vi "Persistent_MakePersistent.vi"(7 "Action":T1=enum."GeneratePattern", 8 "error in (no error)":errorcluster, 10 "DataIn":variant, 11 "ClassRefToActOn":refnum<vi>) -> (0 "error out":errorcluster, 1 "Name":string, 2 "DataOut":variant, 3 "Cancelled":bool)   [LabVIEW 2020]
uses:
  Provider_BaseClassInterface/BaseProvider_SubVIs/BaseProvider_DesignPatternsActions.ctl
  Common/LvClass_class/GDSLvClass_ProviderTypes.ctl
  Provider_EndevoGOOP400/EndevoG4ProviderName.ctl
  <vilib>/picture/picture.llb/imagedata.ctl
  <vilib>/Utility/miscctls.llb/LVPositionTypeDef.ctl
panel:
  in  "StartAsPersitent":bool
  in  "_Cancel":bool
  in  "_OK":bool
  # "Persistent"
  # "This option will add an input to the New.vi that can make the objects persistent."
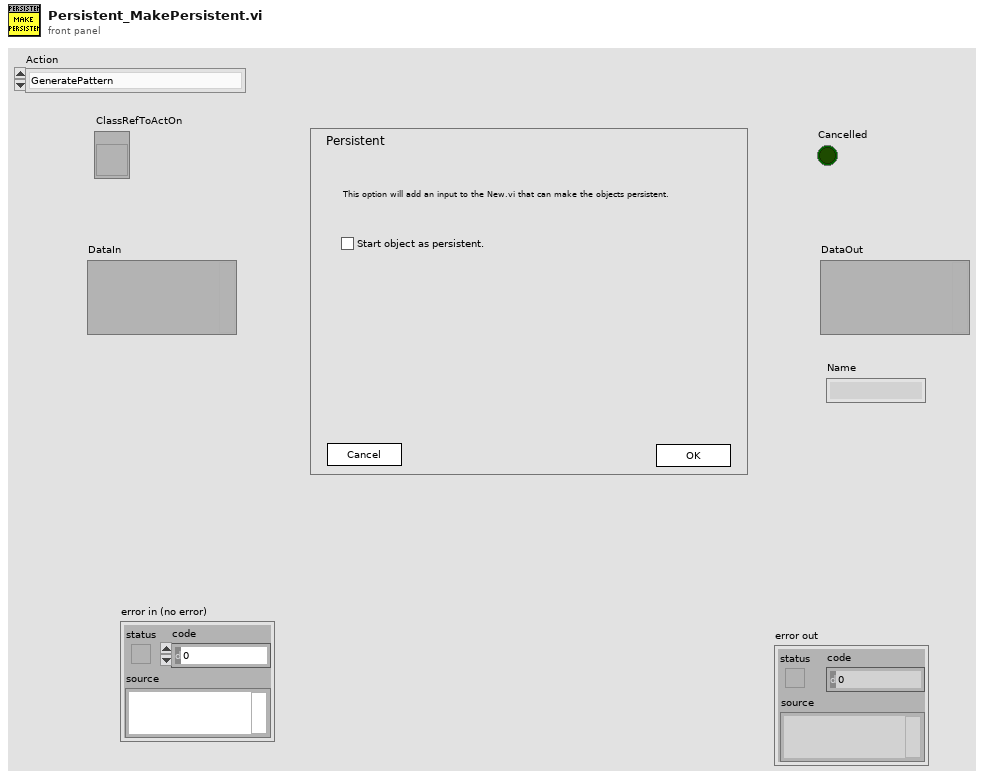
[diagram p1: front panel]
types:
  T1 = typedef "BaseProvider_DesignPatternsActions.ctl" = enum16{"AddPatternDialog", "GeneratePattern", "RemovePattern", "CreatePatternMethod", "UpdatePattern"}
  T2 = typedef "GDSLvClass_ProviderTypes.ctl" = enum16{"UnKnown(LabVOOP)", "Native", "EndevoGOOP3", "OpenG(RootObject)", "OpenG(OpenG_Object)", "EndevoGOOP4", "JKI1"}
  T3 = cluster{"Application":refnum<vi>, "SupportFolder":path, "TemplateName":string, "ClassProvider":T2, "UtilsFolder":path, "UtilsFolderRef":refnum<vi>, "ClassName":string, "Persistent_New.vi":path, "Persistent_CreateReference.vi":path, "NewRef":refnum<vi>, "CreateReferenceRef":refnum<vi>, "ProcessIdRef":refnum<vi>, "TemplateNewRef":refnum<vi>, "StartAsPersitent":bool, "PersistentCPIndex":i32, "FullClassName":string}
  T4 = cluster{"Cancelled":bool, "ClassPath":path, "DataOut":variant, "ClassName":string}
  T5 = typedef "EndevoG4ProviderName.ctl" = enum16{"EndevoGOOP400"}
  T6 = enum32{"invalid lock state", "Not Locked", "Locked (No Password)", "Password-protected"}
  T7 = typedef "LVPositionTypeDef.ctl" = cluster{"Left":i32, "Top":i32}
  T8 = typedef "imagedata.ctl" = cluster{"image type":i32, "image depth":i32, "image":u8[], "mask":u8[], "colors":u32[], "Rectangle":cluster{"left":i16, "top":i16, "right":i16, "bottom":i16}}
  T9 = typedef "GDSLvCLass_ClassSettingsType.ctl" = cluster{"ClassProviderName":string, "ClassTemplateUsed":string, "ClassTemplateVersion":string, "ClassDescription":string, "PlugIns":T10[], "ConnectorPanePattern":string}
  T10 = typedef "GDSLvClass_PlugIn.ctl" = cluster{"Type":T11, "ID":string, "Version":string, "Path":path, "Name":string, "Data":variant}
  T11 = typedef "GDSLvClass_PlugInTypes.ctl" = enum16{"DesignPattern", "MethodTypes"}
  T12 = typedef "GOOP400_Options.ctl" = cluster{"FlatFolderStructure":bool}
  T13 = typedef "GDSLvClass_IconSettingsType.ctl" = cluster{"Frame":u32, "Frame thickness":u8, "Header Background":u32, "Header Text":u32, "ColorPublic":u32, "ColorProtected":u32, "ColorPrivate":u32, "Body Text":u32, "ClassBodyIcon":string}
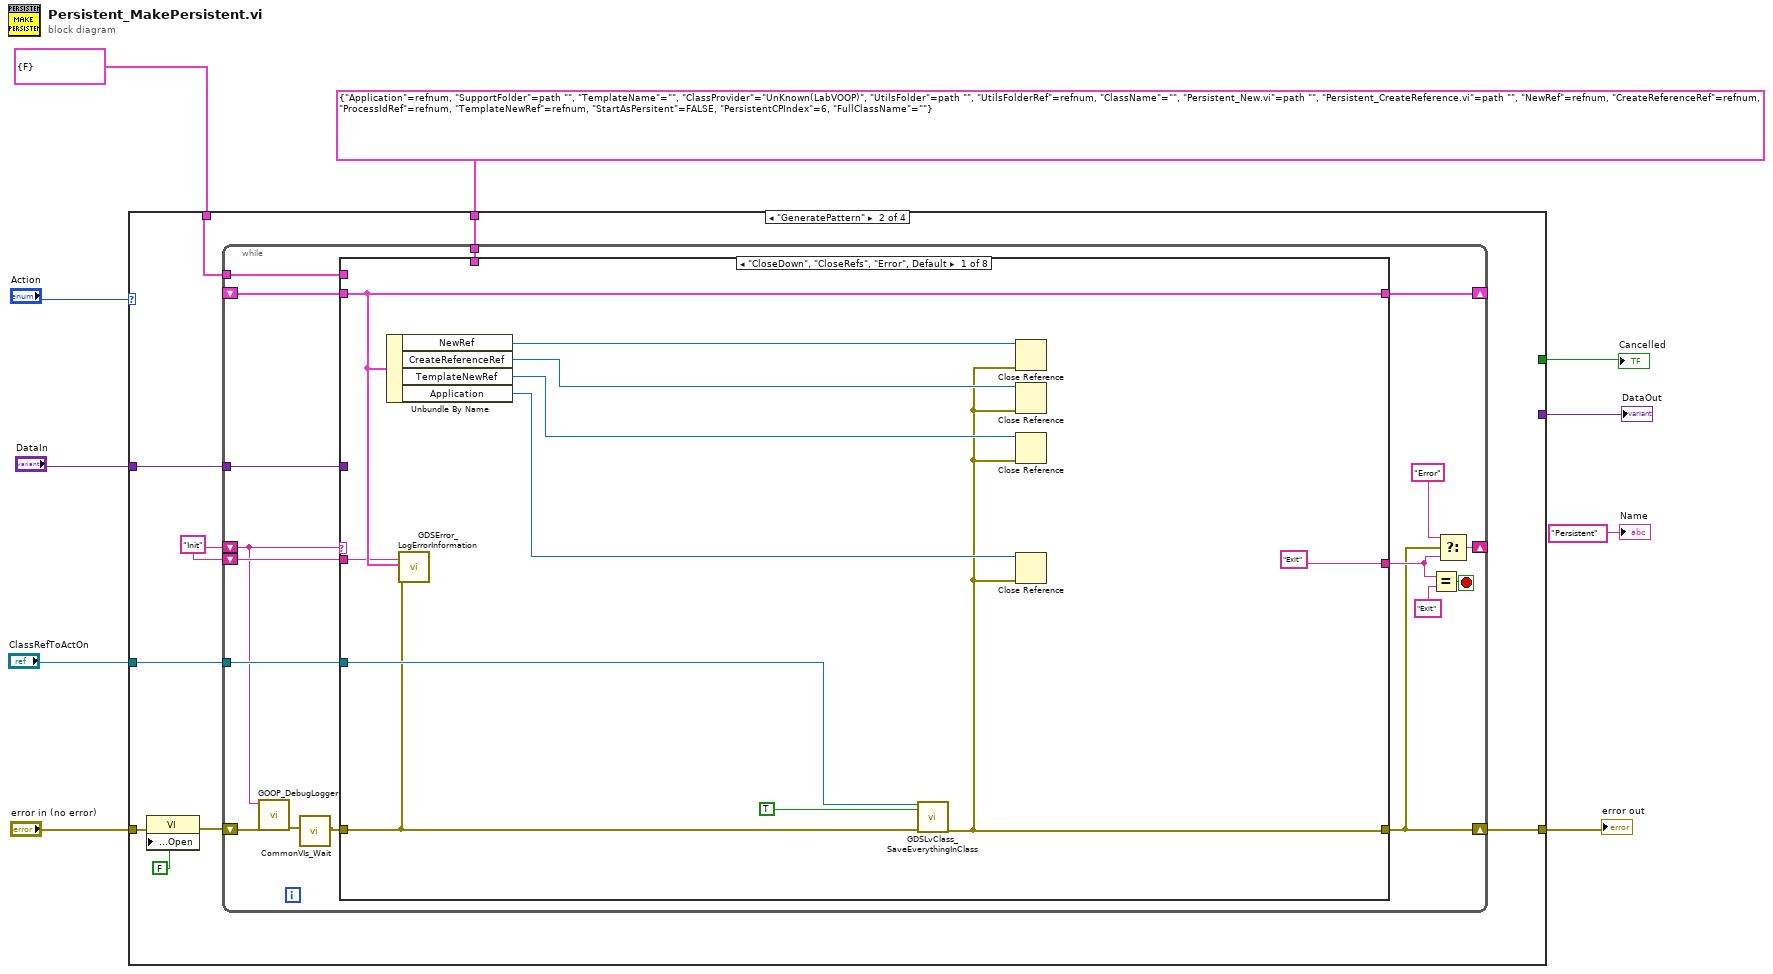
[diagram p0: block diagram]
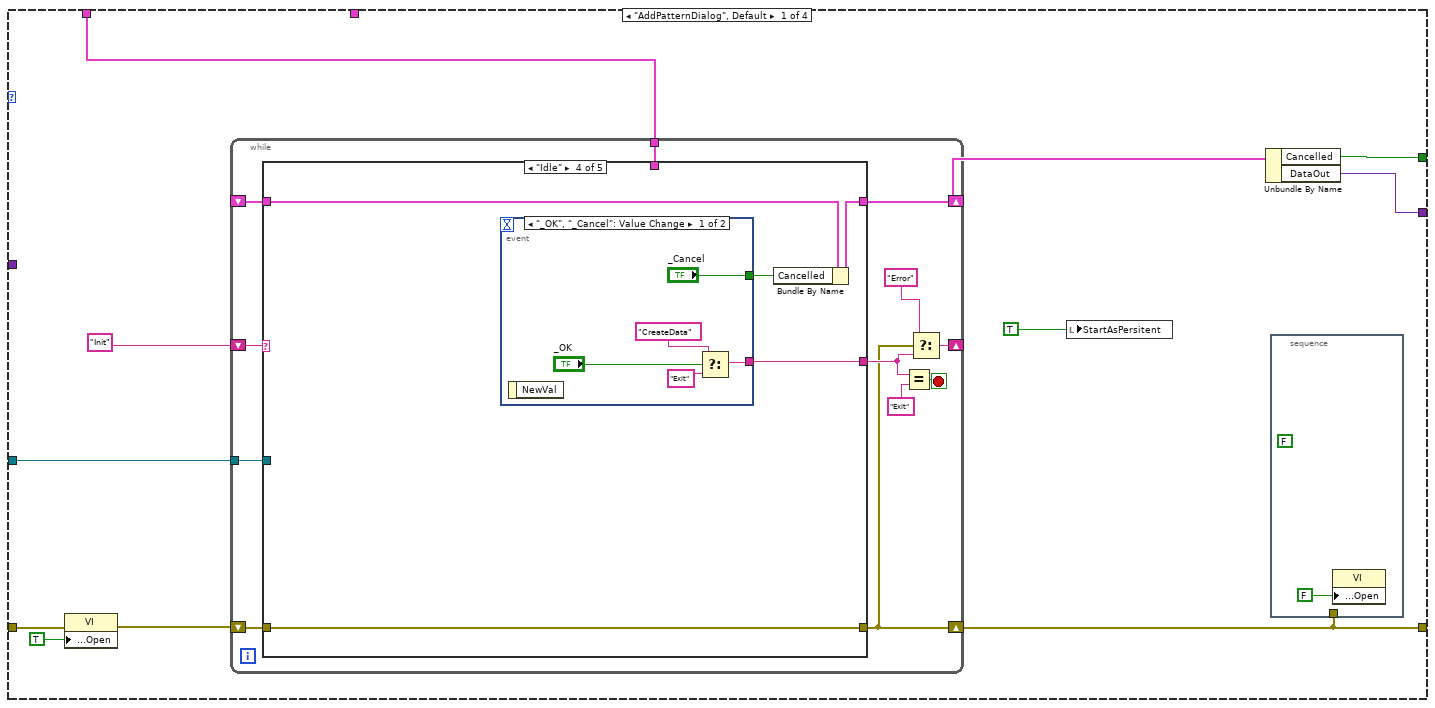
[diagram p2: hidden frame]
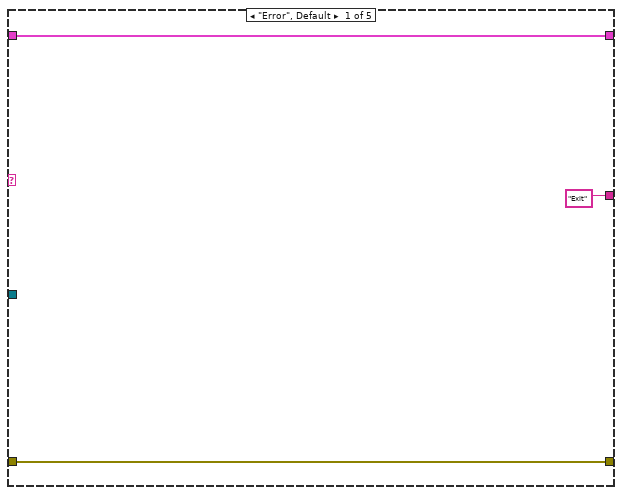
[diagram p3: hidden frame]
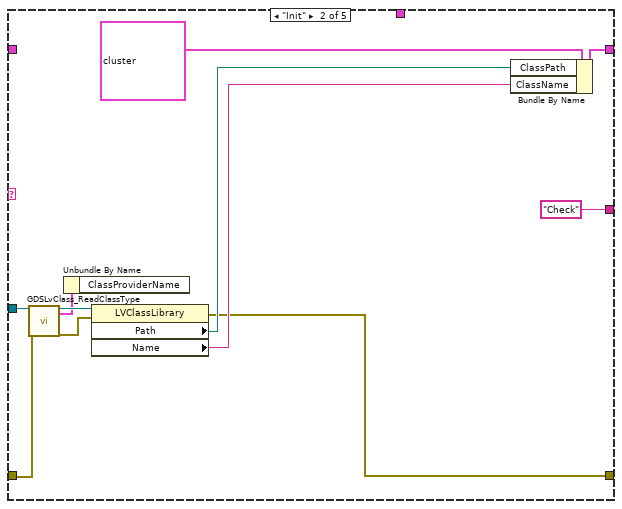
[diagram p4: hidden frame]
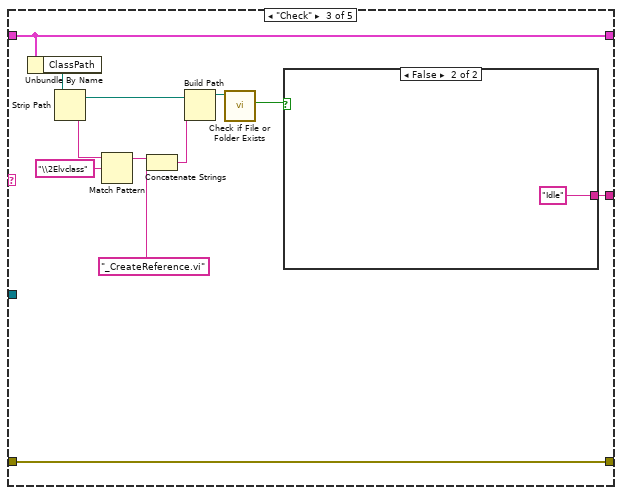
[diagram p5: hidden frame]
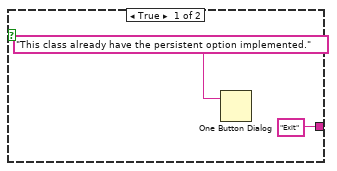
[diagram p6: hidden frame]
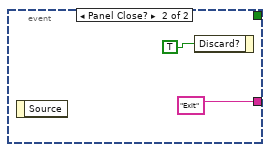
[diagram p7: hidden frame]
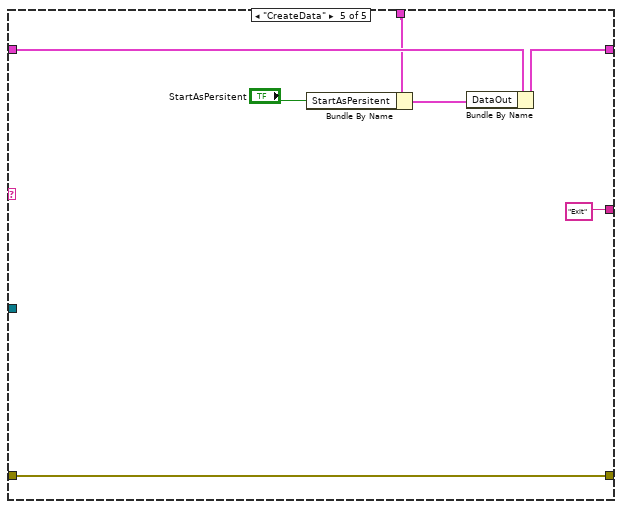
[diagram p8: hidden frame]
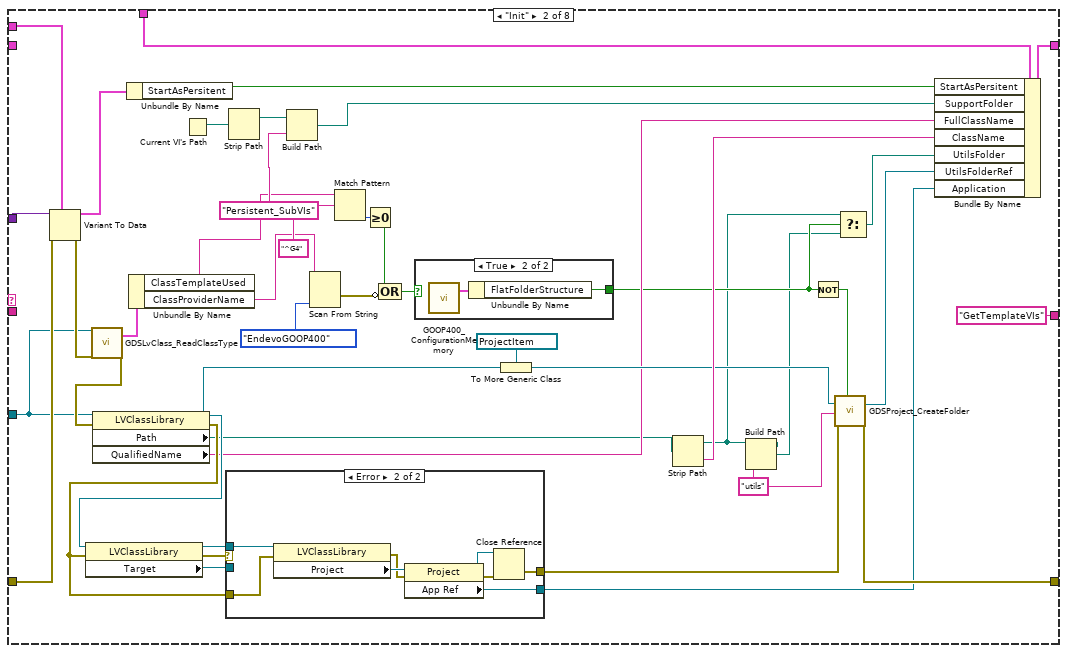
[diagram p9: hidden frame]
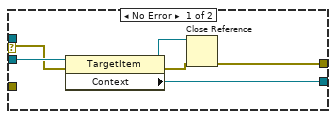
[diagram p11: hidden frame]
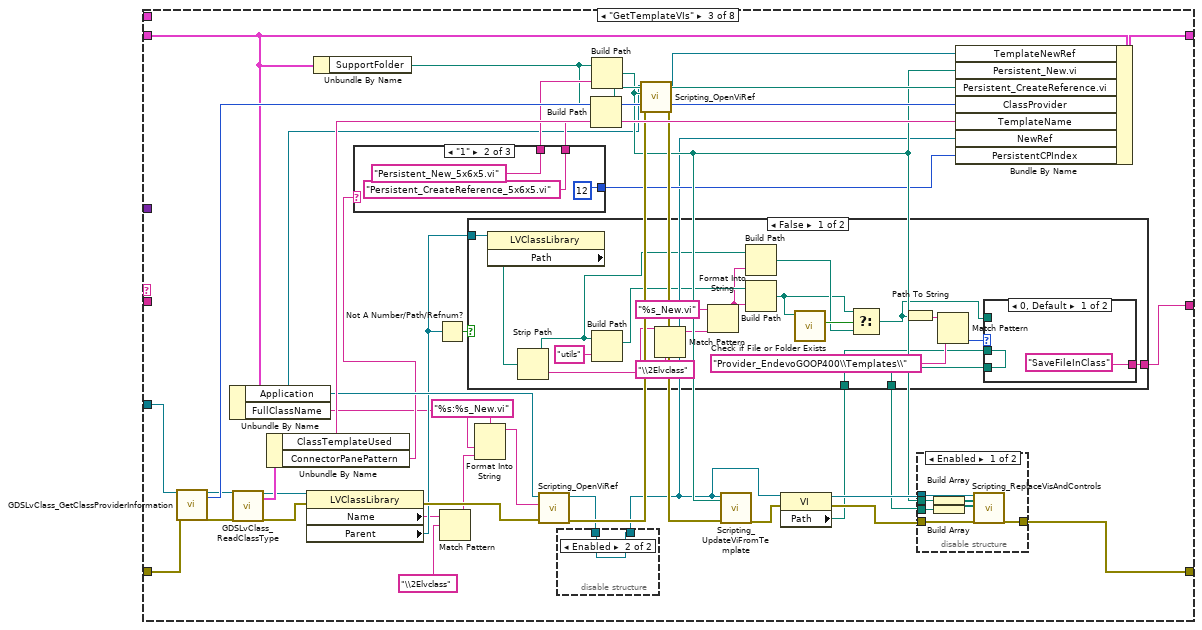
[diagram p12: hidden frame]
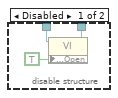
[diagram p13: hidden frame]
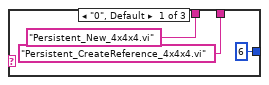
[diagram p14: hidden frame]
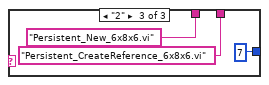
[diagram p15: hidden frame]
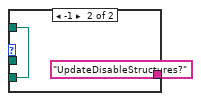
[diagram p16: hidden frame]
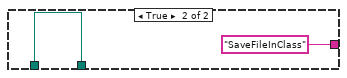
[diagram p17: hidden frame]
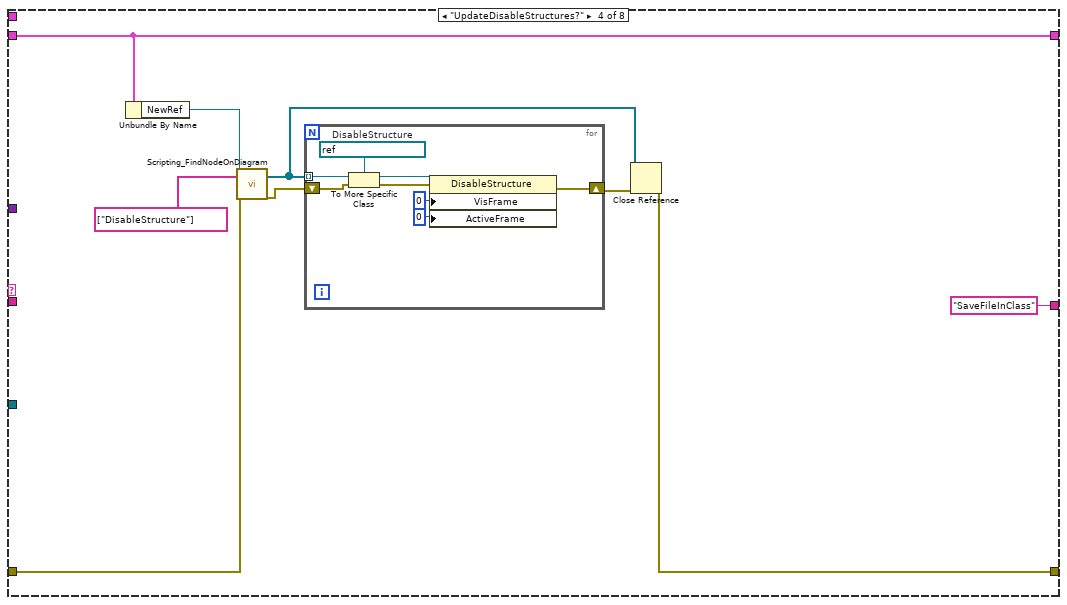
[diagram p19: hidden frame]
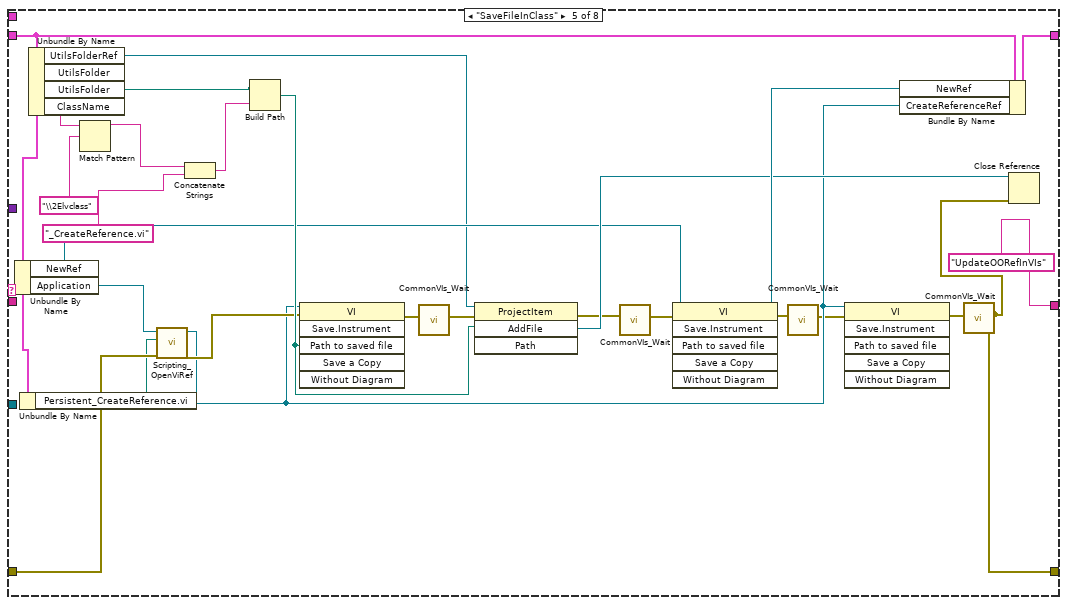
[diagram p20: hidden frame]
diagram:
  n1 = case shown="\"GeneratePattern\"" "Action" {
    tunnel: "error in (no error)" -> [w21 w85 w461 w462]
    tunnel: [w20 w91 w461 w462] -> w8
    tunnel: "ClassRefToActOn" -> [w18 w87 _ _]
    tunnel: [w17 _ _ _] -> w6
    tunnel: [w16 _ _ _] -> w5
    tunnel: cluster{"StartAsPersitent":bool} {"StartAsPersitent"=FALSE} ("output cluster") -> [w15 w89 _ _]
    tunnel: "DataIn" -> [_ w90 _ _]
    tunnel: T3 {"Application"=refnum, "SupportFolder"=path "", "TemplateName"="", "ClassProvider"=enum."UnKnown(LabVOOP)", "UtilsFolder"=path "", "UtilsFolderRef"=refnum, "ClassName"="", "Persistent_New.vi"=path "", "Persistent_CreateReference.vi"=path "", "NewRef"=refnum, "CreateReferenceRef"=refnum, "ProcessIdRef"=refnum, "TemplateNewRef"=refnum, "StartAsPersitent"=FALSE, "PersistentCPIndex"=6, "FullClassName"=""} -> [_ w88 _ _]
    frame "AddPatternDialog", Default {
      n2 = property class="VI"(error in=w21, "Front Panel.Open"=TRUE ("Front Panel Window:Open")) -> (error out=w12:errorcluster)  [unwired: 1 in, 1 out]
      n3 = while {
        shift-right: [w26] -> w20
        shift-left: w12 -> [w33]
        shift-right: [w31] -> _
        shift-left: "Init" -> [w32]
        shift-right: [w25] -> w19
        shift-left: _ -> [w24]
        tunnel: w18 -> [w23]
        tunnel: w15 -> [w22]
        stop <- w30 stop-if-true
        n4 = case shown="\"Idle\"" w32 {
          tunnel: w33 -> [w36 w41 w57 w66 w78]
          tunnel: [w36 w37 w57 w66 w78] -> w26
          tunnel: ["Exit" "Check" w59 w67 "Exit"] -> w27
          tunnel: [w34 w45 w58 w65 w80] -> w25
          tunnel: w24 -> [w34 _ w58 w63 w81]
          tunnel: w23 -> [_ w43 _ _ _]
          tunnel: w22 -> [_ _ _ _ w75]
          frame "Error", Default {
          }
          frame "Init" {
            n5 = call "GDSLvClass_ReadClassType.vi"("Class Refnum In"=w43, "error in (no error)"=w41) -> ("Class Refnum Out"=w42:refnum<vi>, "ClassSettings"=w39:T9, "error out"=w40:errorcluster)  [unwired: 15 in]
            n6 = Unbundle By Name(w39) -> ()  [unwired: 1 out]
            n7 = property class="LVClassLibrary"(reference=w42, error in=w40) -> (error out=w37:errorcluster, "Path"=w44:path, "Name"=w38:string)  [unwired: 1 out]
            n8 = Bundle By Name(cluster=T4 {"Cancelled"=FALSE, "ClassPath"=path "", "DataOut"=variant, "ClassName"=""}, "ClassPath"=w44, "ClassName"=w38) -> (w45:T4)
          }
          frame "Check" {
            n9 = Unbundle By Name(w58) -> ("ClassPath"=w56:path)
            n10 = Strip Path(path=w56) -> (stripped path=w50:path, name=w55:string)
            n11 = Match Pattern(string=w55, regular expression="\\2Elvclass") -> (before substring=w53:string)  [unwired: 1 in, 3 out]
            n12 = Concatenate Strings(w53, "_CreateReference.vi" ("element")) -> (w51:string)
            n13 = Build Path(base path=w50, name or relative path=w51) -> (appended path=w49:path)
            n14 = call <vilib>:"Check if File or Folder Exists.vi"("path"=w49) -> ("file or folder exists?"=w48:bool)  [unwired: 8 in, 2 out]
            n15 = case shown="False" w48 {
              tunnel: ["Exit" "Idle"] -> w59
              frame True {
                n16 = One Button Dialog(message="This class already have the persistent option implemented.") -> ()  [unwired: 1 in, 1 out]
              }
              frame False {
              }
            }
          }
          frame "Idle" {
            n17 = event shown="[0] \"_OK\", \"_Cancel\": Value Change" {
              selector: _ -> [_ _]
              dyn-events: _ -> [_ _]
              timeout: _ -> [_ _]
              tunnel: [w71 "Exit"] -> w67
              tunnel: ["_Cancel" _] -> w64
              event "_OK", "_Cancel": Value Change {
                n18 = event-data() -> ()  [unwired: 1 in, 1 out]
                n19 = Select(t="CreateData", s="_OK", f="Exit") -> (s? t:f=w71:string)
              }
              event Panel Close? {
                n20 = event-data() -> ()  [unwired: 1 in, 1 out]
                n21 = event-data("Discard?"=TRUE) -> ()  [unwired: 1 in, 1 out]
              }
            }
            n22 = Bundle By Name(cluster=w63, "Cancelled"=w64) -> (w65:T4)
          }
          frame "CreateData" {
            n23 = Bundle By Name(cluster=w75, "StartAsPersitent"="StartAsPersitent") -> (w76:cluster{"StartAsPersitent":bool})
            n24 = Bundle By Name(cluster=w81, "DataOut"=w76) -> (w80:T4)
          }
        }
        n25 = Equal?(x=w27, y="Exit") -> (x = y?=w30:bool)
        n26 = Select(t="Error", s=w26, f=w27) -> (s? t:f=w31:string)
      }
      n27 = local write "StartAsPersitent"(TRUE ("StartAsPersitent")) -> ()
      n28 = Unbundle By Name(w19) -> ("Cancelled"=w17:bool, "DataOut"=w16:variant)
      n29 = stacked-sequence {
        tunnel: w20 -> [_]
        frame #0 {
          (unwired) FALSE ("Visible")
          n30 = property class="VI"("Front Panel.Open"=FALSE ("Front Panel Window:Open")) -> ()  [unwired: 2 in, 2 out]
        }
      }
    }
    frame "GeneratePattern" {
      w83 = "Init"
      n31 = property class="VI"(error in=w85, "Front Panel.Open"=FALSE ("Front Panel Window:Open")) -> (error out=w84:errorcluster)  [unwired: 1 in, 1 out]
      n32 = while {
        shift-right: [w103] -> w91
        shift-left: w84 -> [w94]
        shift-right: [w108] -> _
        shift-left: w83 -> [w95]
        shift-right: [w102] -> _
        shift-left: _ -> [w101]
        tunnel: w90 -> [w100]
        tunnel: w89 -> [w99]
        tunnel: w88 -> [w98]
        tunnel: w87 -> [w97]
        shift-left: w83 -> [w96]
        stop <- w107 stop-if-true
        n33 = call "GOOP_DebugLogger.vi"("error in (no error)"=w94, "State"=w95) -> ("error out"=w93:errorcluster)  [unwired: 7 in, 2 out]
        n34 = call "CommonVIs_Wait.vi"("error in"=w93) -> ("error out"=w92:errorcluster)  [unwired: 9 in]
        n35 = case shown="\"CloseDown\", \"CloseRefs\", \"Error\", Default" w95 {
          tunnel: w92 -> [w109 w149 w218 w270 w302 w332 w359 w416]
          tunnel: [w112 w156 w201 w269 w285 w321 w379 w415] -> w103
          tunnel: ["Exit" "GetTemplateVIs" w187 "SaveFileInClass" "UpdateOORefInVIs" w313 "UpdateIcons" "CloseRefs"] -> w104
          tunnel: [w111 w162 w216 w268 w310 w315 w363 w418] -> w102
          tunnel: w101 -> [w111 _ w207 w268 w307 w315 w363 w418]
          tunnel: w100 -> [_ w150 _ _ _ _ _ _]
          tunnel: w99 -> [_ w148 _ _ _ _ _ _]
          tunnel: w98 -> [_ w161 _ _ _ _ _ _]
          tunnel: w97 -> [w115 w121 w219 _ _ w331 _ w420]
          tunnel: w96 -> [w110 _ _ _ _ _ _ _]
          frame "CloseDown", "CloseRefs", "Error", Default {
            n36 = Unbundle By Name(w111) -> ("NewRef"=w118:refnum<vi>, "CreateReferenceRef"=w117:refnum<vi>, "TemplateNewRef"=w114:refnum<vi>, "Application"=w113:refnum<vi>)
            n37 = call "GDSError_LogErrorInformation.vi"("State"=w110, "LocalVariableData"=w111, "error in (no error)"=w109) -> ()  [unwired: 16 in, 1 out]
            n38 = call "GDSLvClass_SaveEverythingInClass.vi"("ClassRefIn"=w115, "ForceResaving(False)"=TRUE, "error in"=w109) -> ("error out"=w112:errorcluster)  [unwired: 15 in, 1 out]
            n39 = Close Reference(reference=w118, error in (no error)=w112) -> ()  [unwired: 1 out]
            n40 = Close Reference(reference=w117, error in (no error)=w112) -> ()  [unwired: 1 out]
            n41 = Close Reference(reference=w114, error in (no error)=w112) -> ()  [unwired: 1 out]
            n42 = Close Reference(reference=w113, error in (no error)=w112) -> ()  [unwired: 1 out]
          }
          frame "Init" {
            w152 = "utils" ("name or relative path")
            n43 = Variant To Data(error in=w149, type=w148, Variant=w150) -> (data=w147:cluster{"StartAsPersitent":bool}, error out=w128:errorcluster)
            n44 = call "GDSLvClass_ReadClassType.vi"("Class Refnum In"=w121, "error in (no error)"=w128) -> ("ClassSettings"=w131:T9, "error out"=w127:errorcluster)  [unwired: 15 in, 1 out]
            n45 = property class="LVClassLibrary"(reference=w121, error in=w127) -> (reference out=w145:refnum<vi>, error out=w139:errorcluster, "Path"=w122:path, "QualifiedName"=w138:string)
            n46 = property class="LVClassLibrary"(reference=w145, error in=w139) -> (reference out=w140:refnum<vi>, error out=w144:errorcluster, "Target"=w143:refnum<vi>)
            n47 = Unbundle By Name(w147) -> ("StartAsPersitent"=w146:bool)
            n48 = Unbundle By Name(w131) -> ("ClassTemplateUsed"=w130:string, "ClassProviderName"=w129:string)
            n49 = Current VI's Path() -> (path=w159:path)
            n50 = case shown="Error" w144 {
              selector: w144 -> [w167 _]
              tunnel: w143 -> [w171 _]
              tunnel: [w170 w173] -> w142
              tunnel: [w166 w174] -> w141
              tunnel: w140 -> [_ w179]
              tunnel: w139 -> [_ w178]
              frame No Error {
                n51 = property class="TargetItem"(reference=w171, error in=w167) -> (reference out=w168:refnum<vi>, error out=w169:errorcluster, "Context"=w170:refnum<vi>)
                n52 = Close Reference(reference=w168, error in (no error)=w169) -> (error out=w166:errorcluster)
              }
              frame Error {
                n53 = property class="LVClassLibrary"(reference=w179, error in=w178) -> (error out=w172:errorcluster, "Project"=w177:refnum<vi>)  [unwired: 1 out]
                n54 = property class="Project"(reference=w177, error in=w172) -> (reference out=w175:refnum<vi>, error out=w176:errorcluster, "App Ref"=w173:refnum<vi>)
                n55 = Close Reference(reference=w175, error in (no error)=w176) -> (error out=w174:errorcluster)
              }
            }
            n56 = Strip Path(path=w159) -> (stripped path=w158:path)  [unwired: 1 out]
            n57 = Build Path(base path=w158, name or relative path="Persistent_SubVIs") -> (appended path=w155:path)
            n58 = Scan From String(input string=w129, default 1=EndevoG4ProviderName."EndevoGOOP400" ("ProviderName")) -> (error out=w135:errorcluster)  [unwired: 4 in, 2 out]
            n59 = Match Pattern(string=w130, regular expression="^G4") -> (offset past match=w134:i32)  [unwired: 1 in, 3 out]
            n60 = Greater Or Equal To 0?(x=w134) -> (x >= 0?=w136:bool)
            n61 = Compound Arithmetic op=OR(w136, invert w135) -> (w137:bool)
            n62 = case shown="True" w137 {
              tunnel: [_ w164] -> w126
              frame False {
              }
              frame True {
                n63 = call "GOOP400_ConfigurationMemory.vi"() -> ("OptionsOut"=w165:T12)  [unwired: 18 in, 1 out]
                n64 = Unbundle By Name(w165) -> ("FlatFolderStructure"=w164:bool)
              }
            }
            n65 = To More Generic Class(target class=refnum<vi> refnum ("AddItem"), reference=w145) -> (generic class reference=w151:refnum<vi>)
            n66 = Strip Path(path=w122) -> (stripped path=w125:path, name=w153:string)
            n67 = Build Path(base path=w125, name or relative path=w152) -> (appended path=w124:path)
            n68 = Not(x=w126) -> (.not. x?=w120:bool)
            n69 = call "GDSProject_CreateFolder.vi"("Project Item To Create Folder Below(Use MyComputer if not wired)"=w151, "FolderName"=w152, "error in (no error)"=w141, "CreateThePhysicalFolderIfPossible(False)"=w120) -> ("ItemOut"=w154:refnum<vi>, "error out"=w156:errorcluster)  [unwired: 12 in, 2 out]
            n70 = Select(t=w125, s=w126, f=w124) -> (s? t:f=w123:path)
            n71 = Bundle By Name(cluster=w161, "StartAsPersitent"=w146, "SupportFolder"=w155, "FullClassName"=w138, "ClassName"=w153, "UtilsFolder"=w123, "UtilsFolderRef"=w154, "Application"=w142) -> (w162:T3)
          }
          frame "GetTemplateVIs" {
            n72 = call "GDSLvClass_GetClassProviderInformation.vi"("Class Refnum In"=w219, "error in (no error)"=w218) -> ("Class Refnum Out"=w215:refnum<vi>, "ClassProvider"=w217:T2, "error out"=w214:errorcluster)  [unwired: 15 in]
            n73 = Unbundle By Name(w207) -> ("Application"=w189:refnum<vi>, "FullClassName"=w183:string)
            n74 = call "GDSLvClass_ReadClassType.vi"("Class Refnum In"=w215, "error in (no error)"=w214) -> ("Class Refnum Out"=w195:refnum<vi>, "ClassSettings"=w213:T9, "error out"=w194:errorcluster)  [unwired: 15 in]
            n75 = Unbundle By Name(w213) -> ("ClassTemplateUsed"=w212:string, "ConnectorPanePattern"=w186:string)
            n76 = property class="LVClassLibrary"(reference=w195, error in=w194) -> (error out=w193:errorcluster, "Name"=w184:string, "Parent"=w188:refnum<vi>)  [unwired: 1 out]
            n77 = Unbundle By Name(w207) -> ("SupportFolder"=w210:path)
            n78 = case shown="\"1\"" w186 {
              tunnel: ["Persistent_New_4x4x4.vi" ("name or relative path") "Persistent_New_5x6x5.vi" ("name or relative path") "Persistent_New_6x8x6.vi" ("name or relative path")] -> w211
              tunnel: ["Persistent_CreateReference_4x4x4.vi" ("name or relative path") "Persistent_CreateReference_5x6x5.vi" ("name or relative path") "Persistent_CreateReference_6x8x6.vi" ("name or relative path")] -> w209
              tunnel: [6 ("PersistentCPIndex") 12 ("PersistentCPIndex") 7 ("PersistentCPIndex")] -> w185
              frame "0", Default {
              }
              frame "1" {
              }
              frame "2" {
              }
            }
            n79 = Not A Number/Path/Refnum?(number/path/refnum=w188) -> (NaN/Path/Refnum?=w192:bool)
            n80 = Match Pattern(string=w184, regular expression="\\2Elvclass") -> (before substring=w182:string)  [unwired: 1 in, 3 out]
            n81 = Format Into String(format string="%s:%s_New.vi", w183, w182) -> (resulting string=w204:string)  [unwired: 2 in, 1 out]
            n82 = call "Scripting_OpenViRef.vi"("error in"=w193, "ViPath/ViName/Viref"=w204, "AppRef"=w189) -> ("error out"=w199:errorcluster, "vi reference"=w181:refnum<vi>)  [unwired: 6 in, 1 out]
            n83 = disable-structure shown="Enabled" {
              disable-tunnel: w181 -> [w221 w223]
              disable-tunnel: [w220 w223] -> w180
              frame Disabled {
                n84 = property class="VI"(reference=w221, "BDWin.Open"=TRUE ("Block Diagram Window:Open")) -> (reference out=w220:refnum<vi>)  [unwired: 1 in, 1 out]
              }
              frame Enabled {
              }
            }
            n85 = Build Path(base path=w210, name or relative path=w209) -> (appended path=w208:path)
            n86 = Build Path(base path=w210, name or relative path=w211) -> (appended path=w197:path)
            n87 = call "Scripting_OpenViRef.vi"("error in"=w199, "ViPath/ViName/Viref"=w197, "AppRef"=w189) -> ("error out"=w198:errorcluster, "vi reference"=w196:refnum<vi>)  [unwired: 6 in, 1 out]
            n88 = call "Scripting_UpdateViFromTemplate.vi"("ViRef"=w180, "TemplateVI(Path or Ref)"=w197, "error in (no error)"=w198) -> ("error out"=w200:errorcluster)  [unwired: 15 in, 1 out]
            n89 = property class="VI"(reference=w180, error in=w200) -> (reference out=w203:refnum<vi>, error out=w202:errorcluster, "Path"=w191:path)
            n90 = case shown="False" w192 {
              tunnel: [w240 w258] -> w190
              tunnel: w191 -> [w239 w258]
              tunnel: w188 -> [w252 _]
              tunnel: [w244 "SaveFileInClass"] -> w187
              frame False {
                n91 = property class="LVClassLibrary"(reference=w252) -> ("Path"=w249:path)  [unwired: 1 in, 2 out]
                n92 = Strip Path(path=w249) -> (stripped path=w237:path, name=w248:string)
                n93 = Build Path(base path=w237, name or relative path="utils") -> (appended path=w246:path)
                n94 = Match Pattern(string=w248, regular expression="\\2Elvclass") -> (before substring=w245:string)  [unwired: 1 in, 3 out]
                n95 = Format Into String(format string="%s_New.vi", w245) -> (resulting string=w236:string)  [unwired: 2 in, 1 out]
                n96 = Build Path(base path=w237, name or relative path=w236) -> (appended path=w235:path)
                n97 = Build Path(base path=w246, name or relative path=w236) -> (appended path=w234:path)
                n98 = call <vilib>:"Check if File or Folder Exists.vi"("path"=w234) -> ("file or folder exists?"=w238:bool)  [unwired: 8 in, 2 out]
                n99 = Select(t=w234, s=w238, f=w235) -> (s? t:f=w233:path)
                n100 = Path To String(path=w233) -> (string=w243:string)
                n101 = Match Pattern(string=w243, regular expression="Provider_EndevoGOOP400\\Templates\\") -> (offset past match=w241:i32)  [unwired: 1 in, 3 out]
                n102 = case shown="0, Default" w241 {
                  tunnel: ["SaveFileInClass" "UpdateDisableStructures?"] -> w244
                  tunnel: [w253 w255] -> w240
                  tunnel: w233 -> [_ w255]
                  tunnel: w239 -> [w253 _]
                  frame 0, Default {
                  }
                  frame -1 {
                  }
                }
              }
              frame True {
              }
            }
            n103 = disable-structure shown="Enabled" {
              disable-tunnel: w202 -> [w265 w266]
              disable-tunnel: [w264 w266] -> w201
              disable-tunnel: w203 -> [w263 _]
              disable-tunnel: w190 -> [w260 _]
              disable-tunnel: w197 -> [w259 _]
              frame Enabled {
                n104 = Build Array(w259) -> (w262:path[])
                n105 = Build Array(w260) -> (w261:path[])
                n106 = call "Scripting_ReplaceVisAndControls.vi"("ViRef"=w263, "OldVIsAndControls"=w262, "NewVIsAndControls"=w261, "error in (no error)"=w265) -> ("error out"=w264:errorcluster)  [unwired: 15 out]
              }
              frame Disabled {
              }
            }
            n107 = Bundle By Name(cluster=w207, "TemplateNewRef"=w196, "Persistent_New.vi"=w197, "Persistent_CreateReference.vi"=w208, "ClassProvider"=w217, "TemplateName"=w212, "NewRef"=w180, "PersistentCPIndex"=w185) -> (w216:T3)
          }
          frame "UpdateDisableStructures?" {
            n108 = Unbundle By Name(w268) -> ("NewRef"=w267:refnum<vi>)
            n109 = call "Scripting_FindNodeOnDiagram.vi"("ViRef(Ignored If Not Wired)"=w267, "NodeTypesToSearchFor"=string[] ["DisableStructure"], "error in (no error)"=w270) -> ("Nodes"=w271:refnum<vi>[], "error out"=w273:errorcluster)  [unwired: 15 in]
            n110 = for {
              tunnel: w271 -> [w283] mode=indexing
              shift-right: [w276] -> w272
              shift-left: w273 -> [w281]
              w282 = refnum<vi> refnum  # DisableStructure
              n111 = To More Specific Class(target class=w282, reference=w283, error in=w281) -> (specific class reference=w278:refnum<vi>, error out=w279:errorcluster)
              n112 = property class="DisableStructure"(reference=w278, error in=w279, "VisFrame"=u32 0 ("Visible Frame"), "ActiveFrame"=i16 0 ("Active Frame")) -> (error out=w276:errorcluster)  [unwired: 1 out]
            }
            n113 = Close Reference(reference=w271, error in (no error)=w272) -> (error out=w269:errorcluster)
          }
          frame "SaveFileInClass" {
            n114 = Unbundle By Name(w307) -> ("NewRef"=w294:refnum<vi>, "Application"=w298:refnum<vi>)
            n115 = Unbundle By Name(w307) -> ("Persistent_CreateReference.vi"=w299:path)
            n116 = Unbundle By Name(w307) -> ("UtilsFolderRef"=w293:refnum<vi>, "UtilsFolder"=w284:path, "ClassName"=w306:string)  [unwired: 1 out]
            n117 = Match Pattern(string=w306, regular expression="\\2Elvclass") -> (before substring=w297:string)  [unwired: 1 in, 3 out]
            n118 = call "Scripting_OpenViRef.vi"("error in"=w302, "ViPath/ViName/Viref"=w299, "AppRef"=w298) -> ("error out"=w301:errorcluster, "vi reference"=w300:refnum<vi>)  [unwired: 6 in, 1 out]
            n119 = Concatenate Strings(w297, "_CreateReference.vi" ("name or relative path")) -> (w295:string)
            n120 = Build Path(base path=w284, name or relative path=w295) -> (appended path=w304:path)
            n121 = invoke class="VI" method="Save.Instrument"(reference=w300, error in=w301, "Path to saved file"=w304) -> (error out=w290:errorcluster)  [unwired: 3 in, 5 out]
            n122 = call "CommonVIs_Wait.vi"("error in"=w290) -> ("error out"=w289:errorcluster)  [unwired: 9 in]
            n123 = invoke class="ProjectItem" method="AddFile"(reference=w293, error in=w289, "Path"=w304) -> (error out=w292:errorcluster, "AddFile"=w303:refnum<vi>)  [unwired: 1 in, 2 out]
            n124 = call "CommonVIs_Wait.vi"("error in"=w292) -> ("error out"=w291:errorcluster)  [unwired: 9 in]
            n125 = invoke class="VI" method="Save.Instrument"(reference=w294, error in=w291) -> (reference out=w309:refnum<vi>, error out=w288:errorcluster)  [unwired: 4 in, 4 out]
            n126 = call "CommonVIs_Wait.vi"("error in"=w288) -> ("error out"=w287:errorcluster)  [unwired: 9 in]
            n127 = invoke class="VI" method="Save.Instrument"(reference=w300, error in=w287) -> (error out=w286:errorcluster)  [unwired: 4 in, 5 out]
            n128 = Bundle By Name(cluster=w307, "NewRef"=w309, "CreateReferenceRef"=w300) -> (w310:T3)
            n129 = call "CommonVIs_Wait.vi"("error in"=w286) -> ("error out"=w285:errorcluster)  [unwired: 9 in]
            n130 = Close Reference(reference=w303, error in (no error)=w285) -> ()  [unwired: 1 out]
          }
          frame "UpdateOORefInVIs" {
            (unwired) "UpdateNew"
            n131 = Unbundle By Name(w315) -> ("Persistent_New.vi"=w320:path, "NewRef"=w328:refnum<vi>, "CreateReferenceRef"=w317:refnum<vi>)
            n132 = Unbundle By Name(w315) -> ("StartAsPersitent"=w314:bool)
            n133 = property class="LVClassLibrary"(reference=w331) -> ("Path"=w318:path)  [unwired: 1 in, 2 out]
            n134 = Path To String(path=w318) -> (string=w329:string)
            n135 = Build Array(w318, w318) -> (w316:path[])
            n136 = Build Array(w328, w317) -> (w330:refnum<vi>[])
            n137 = for {
              tunnel: w330 -> [w344] mode=indexing
              shift-right: [w347] -> w322
              shift-left: w332 -> [w346]
              tunnel: w329 -> [w345]
              tunnel: w318 -> [w343]
              tunnel: path[] [path "LabVIEWClassControl", path "LabVIEWClassConstant"] ("OldVIsAndControls") -> [w342]
              tunnel: w316 -> [w341]
              n138 = disable-structure shown="Enabled" {
                disable-tunnel: [w351 w355] -> w347
                disable-tunnel: w346 -> [w350 w356]
                disable-tunnel: w345 -> [w349 _]
                disable-tunnel: w344 -> [w348 w353]
                disable-tunnel: w343 -> [_ _]
                disable-tunnel: w342 -> [_ w354]
                disable-tunnel: w341 -> [_ w352]
                frame Disabled {
                  n139 = call "Scripting_ReplaceOORef.vi"("ViRef"=w348, "NewLvClassFile(ProjectPath or LvClassPath)"=w349, "error in (no error)"=w350) -> ("error out"=w351:errorcluster)  [unwired: 16 in]
                }
                frame Enabled {
                  n140 = call "Scripting_ReplaceVisAndControls.vi"("ViRef"=w353, "OldVIsAndControls"=w354, "NewVIsAndControls"=w352, "error in (no error)"=w356) -> ("error out"=w355:errorcluster)  [unwired: 15 out]
                }
              }
            }
            n141 = invoke class="VI" method="Lock State.Set"(reference=w328, error in=w322, "lockState"=T6."Not Locked" ("Lock State")) -> (reference out=w324:refnum<vi>, error out=w323:errorcluster)  [unwired: 4 in, 5 out]
            n142 = property class="VI"(reference=w324, error in=w323) -> (error out=w326:errorcluster, "Path"=w325:path)  [unwired: 1 out]
            n143 = disable-structure shown="Enabled" {
              disable-tunnel: w326 -> [w339 w340]
              disable-tunnel: [w338 w340] -> w321
              disable-tunnel: w317 -> [w337 _]
              disable-tunnel: w325 -> [w334 _]
              disable-tunnel: w320 -> [w333 _]
              frame Enabled {
                n144 = Build Array(w333) -> (w336:path[])
                n145 = Build Array(w334) -> (w335:path[])
                n146 = call "Scripting_ReplaceVisAndControls.vi"("ViRef"=w337, "OldVIsAndControls"=w336, "NewVIsAndControls"=w335, "error in (no error)"=w339) -> ("error out"=w338:errorcluster)  [unwired: 15 out]
              }
              frame Disabled {
              }
            }
            n147 = Select(t="UpdateCreate", s=w314, f="UpdateIcons") -> (s? t:f=w313:string)
          }
          frame "UpdateCreate" {
            n148 = Unbundle By Name(w363) -> ("NewRef"=w397:refnum<vi>, "Application"=w398:refnum<vi>, "FullClassName"=w360:string, "ClassName"=w378:string)
            n149 = Unbundle By Name(w363) -> ("TemplateName"=w371:string)
            n150 = To Lower Case(string=w371) -> (all lower case string=w370:string)
            n151 = Match Pattern(string=w370, regular expression="singleton") -> (offset past match=w368:i32)  [unwired: 1 in, 3 out]
            n152 = Match Pattern(string=w378, regular expression="\\2Elvclass") -> (before substring=w400:string)  [unwired: 1 in, 3 out]
            n153 = Greater Or Equal To 0?(x=w368) -> (x >= 0?=w367:bool)
            n154 = Select(t="%s:%s_GetInstance.vi" ("format string"), s=w367, f="%s:%s_Create.vi" ("format string")) -> (s? t:f=w364:string)
            n155 = Format Into String(format string=w364, w360, w400) -> (resulting string=w399:string)  [unwired: 2 in, 1 out]
            n156 = call "Scripting_OpenViRef.vi"("error in"=w359, "ViPath/ViName/Viref"=w399, "AppRef"=w398) -> ("error out"=w393:errorcluster, "vi reference"=w358:refnum<vi>)  [unwired: 6 in, 1 out]
            n157 = disable-structure shown="Enabled" {
              disable-tunnel: w358 -> [w403 w405]
              disable-tunnel: [w402 w405] -> w357
              frame Disabled {
                n158 = property class="VI"(reference=w403, "BDWin.Open"=TRUE ("Block Diagram Window:Open")) -> (reference out=w402:refnum<vi>)  [unwired: 1 in, 1 out]
              }
              frame Enabled {
              }
            }
            n159 = property class="VI"(reference=w397, error in=w393) -> (error out=w394:errorcluster, "Path"=w396:path)  [unwired: 1 out]
            n160 = Build Array(w396) -> (w395:path[])
            n161 = call "Scripting_FindVisOnDiagram.vi"("ViRef"=w357, "VIsToSerachFor/ViName"=w395, "error in (no error)"=w394) -> ("VisFound"=w382:refnum<vi>[], "error out"=w391:errorcluster)  [unwired: 15 in]
            n162 = Unbundle By Name(w363) -> ("PersistentCPIndex"=w362:i32)
            n163 = Index Array(array=w382) -> (element=w390:refnum<vi>)  [unwired: 1 in]
            n164 = To More Specific Class(target class=refnum<vi> refnum ("WhileLoop"), reference=w390, error in=w391) -> (specific class reference=w389:refnum<vi>, error out=w388:errorcluster)
            n165 = property class="SubVI"(reference=w389, error in=w388) -> (error out=w386:errorcluster, "Terms[]"=w387:refnum<vi>[])  [unwired: 1 out]
            n166 = Delete From Array(array=w387, index=w362) -> (deleted portion=w375:refnum<vi>, array with subset deleted=w376:refnum<vi>[])  [unwired: 1 in]
            n167 = Close Reference(reference=w376, error in (no error)=w386) -> (error out=w374:errorcluster)
            n168 = invoke class="Term" method="Create Constant"(reference=w375, error in=w374, "Value"=enum16{"Default", "Persistent", "NonPersistent"}."Persistent" ("Persistent/Debugging(Default)")) -> (reference out=w383:refnum<vi>, error out=w385:errorcluster, "Create Constant"=w373:refnum<vi>)  [unwired: 1 in, 1 out]
            n169 = disable-structure shown="Enabled" {
              disable-tunnel: w373 -> [w410 w412]
              disable-tunnel: [w409 w412] -> w372
              frame Disabled {
                n170 = property class="Const"(reference=w410) -> (reference out=w411:refnum<vi>, "Position"=w408:T7)  [unwired: 1 in, 1 out]
                n171 = Add(x=w408, y=T7 {"Left"=0, "Top"=16}) -> (x+y=w407:T7)
                n172 = property class="Const"(reference=w411, "Position"=w407) -> (reference out=w409:refnum<vi>)  [unwired: 1 in, 1 out]
              }
              frame Enabled {
              }
            }
            n173 = Close Reference(reference=w372, error in (no error)=w385) -> (error out=w384:errorcluster)
            n174 = Close Reference(reference=w383, error in (no error)=w384) -> (error out=w380:errorcluster)
            n175 = Close Reference(reference=w382, error in (no error)=w380) -> (error out=w381:errorcluster)
            n176 = Close Reference(reference=w357, error in (no error)=w381) -> (error out=w379:errorcluster)
          }
          frame "UpdateIcons" {
            w437 = u8 32 ("x")
            n177 = Unbundle By Name(w418) -> ("CreateReferenceRef"=w419:refnum<vi>, "NewRef"=w413:refnum<vi>)
            n178 = property class="LVClassLibrary"(reference=w420, error in=w416) -> (reference out=w425:refnum<vi>, error out=w421:errorcluster, "Member Data"=w423:refnum<vi>)
            n179 = call "GDSLvIcon_AnalyseViIcon.vi"("ViRef/LvCLassRef/LvLibRef/ViPath/2D_Image"=w423, "error in (no error)"=w421) -> ("HeaderIcon"=w426:u8[][], "error out"=w422:errorcluster)  [unwired: 5 in, 11 out]
            n180 = disable-structure shown="Enabled" {
              disable-tunnel: w419 -> [w444 w446]
              disable-tunnel: [w443 w445] -> w414
              disable-tunnel: w413 -> [w442 _]
              frame Disabled {
                n181 = Build Array(w444, w442) -> (w443:refnum<vi>[])
              }
              frame Enabled {
                n182 = Build Array(w446) -> (w445:refnum<vi>[])
              }
            }
            n183 = Close Reference(reference=w423, error in (no error)=w422) -> (error out=w424:errorcluster)
            n184 = Array Size(array=w426) -> (size(s)=w432:i32[])
            n185 = call "GDSLvClass_ReadClassColors.vi"("Library Refnum"=w425, "error in (no error)"=w424) -> ("LvClassIconSettings"=w428:T13, "error out"=w417:errorcluster)  [unwired: 12 in, 4 out]
            n186 = Unbundle By Name(w428) -> ("Frame"=w431:u32, "Body Text"=w430:u32, "Frame thickness"=w427:u8)
            n187 = Unbundle By Name(w428) -> ("ColorProtected"=w429:u32)
            n188 = Index Array(array=w432) -> (element #1=w434:i32)  [unwired: 2 in, 1 out]
            n189 = Multiply(x=w427, y=u8 2) -> (x*y=w435:u8)
            n190 = Add(x=w434, y=w435) -> (x+y=w436:i32)
            n191 = Increment(x=w436) -> (x+1=w438:i32)
            n192 = Subtract(x=w437, y=w438) -> (x-y=w439:i32)
            n193 = Subtract(x=w437, y=w435) -> (x-y=w440:u8)
            n194 = for {
              tunnel: w440 -> [_]
              tunnel: w439 -> [_]
              tunnel: w431 -> [w460]
              tunnel: w430 -> [_]
              tunnel: w429 -> [_]
              tunnel: w427 -> [w459]
              tunnel: w426 -> [w458]
              shift-right: [w451] -> w415
              shift-left: w417 -> [w450]
              tunnel: w414 -> [w447] mode=indexing
              n195 = call "GDSLvIcon_AnalyseViIcon.vi"("ViRef/LvCLassRef/LvLibRef/ViPath/2D_Image"=w447, "error in (no error)"=w450) -> ("BodyIcon"=w448:u8[][], "error out"=w449:errorcluster)  [unwired: 5 in, 11 out]
              n196 = call "GDSLvIcon_CreateIconPicture.vi"("FrameColor"=w460, "FrameThickness(1)"=w459, "HeaderIconIn"=w458, "BodyIconIn"=w448, "error in (no error)"=w449) -> ("WholeIconOut"=w453:u8[][], "error out"=w456:errorcluster)  [unwired: 9 in, 4 out]
              n197 = Reshape Array(w453, 1024 ("dimension size")) -> (w455:u8[])
              n198 = Bundle By Name(cluster=T8 {"image type"=0, "image depth"=8, "image"=[], "mask"=[], "colors"=[], "Rectangle"={"left"=0, "top"=0, "right"=32, "bottom"=32}} ("image data"), "image"=w455) -> (w457:T8)
              n199 = invoke class="VI" method="VI Icon.Set from Image Data"(reference=w447, error in=w456, "ImageData"=w457) -> (error out=w451:errorcluster)  [unwired: 3 in, 5 out]
            }
          }
        }
        n200 = Equal?(x=w104, y="Exit") -> (x = y?=w107:bool)
        n201 = Select(t="Error", s=w103, f=w104) -> (s? t:f=w108:string)
      }
    }
    frame "RemovePattern" {
    }
    frame "CreatePatternMethod" {
    }
  }
  "error out" <- w8
  "DataOut" <- w5
  "Cancelled" <- w6
  "Name" <- "Persistent" ("Name")
